vi "Add Process.vi"(8 "error in (no error)":errorcluster, 10 "Process":refnum<class "Process.lvclass">, 11 "Application In":refnum<class "Application.lvclass">) -> (0 "error out":errorcluster, 3 "Application Out":refnum<class "Application.lvclass">)   [LabVIEW 2020, in "Application.lvclass"]
doc: "Add a process to the application. The process should be initialized before being added to the application. After adding a proess, the lifecycle of the process is owned and managed by the owning application. It is therefore not necessary to Start, Stop, or Clear added processes through the lifecycle of the application."
uses:
  Application.lvclass
  C:/git/astemes-triarc-framework/source/Framework/Process/Process.lvclass
  Process/Process.lvclass
  C:/git/astemes-triarc-framework/source/Framework/Logging/Logging.lvclass
  Process/Public/Lifecycle/Lifecycle State.ctl
  Process/Process.lvclass/Process.ctl
  Application.lvclass/Application.ctl
  Synchronous Request Callback/Synchronous Request Callback.lvclass/Synchronous Request Callback.ctl
  Get Process.vi
  Process/Private/SubVIs/Handle Debug Data.vi
  <vilib>/Utility/error.llb/Clear Errors.vi
  Private/Retrieve Process from App.vi
  Private/Parse Process Name.vi
  Private/Get Process from Map.vi
  Logging/Log Debug.vi
  <vilib>/AdvancedString/1D String Array to Delimited String.vi
  <vilib>/Utility/High Resolution Relative Seconds.vi
  Process/Protected/Messaging/Request Message.vi
  <vilib>/AdvancedString/Delimited String to 1D String Array.vi
  Synchronous Request Callback/Create.vi
  Process/Protected/Messaging/Async Request Message.vi
  Synchronous Request Callback/Synchronous Request Callback.lvclass
  C:/git/astemes-triarc-framework/source/Framework/Callback/Callback.lvclass
  <vilib>/Utility/error.llb/Error Cluster From Error Code.vi
  Process/Private/SubVIs/Wait for Response Message.vi
  <vilib>/ErrorRing/Error Ring.xnode
  Callback/Callback.lvclass
  Logging/Logging.lvclass
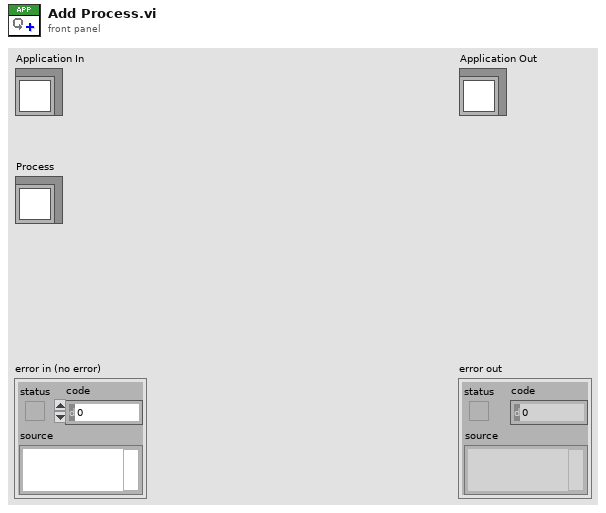
[diagram p1: front panel]
types:
  T1 = typedef "Process.lvclass/Lifecycle State.ctl" = enum16{"Uninitialized", "Initialized", "Started", "Running", "Stopped", "Finished"}
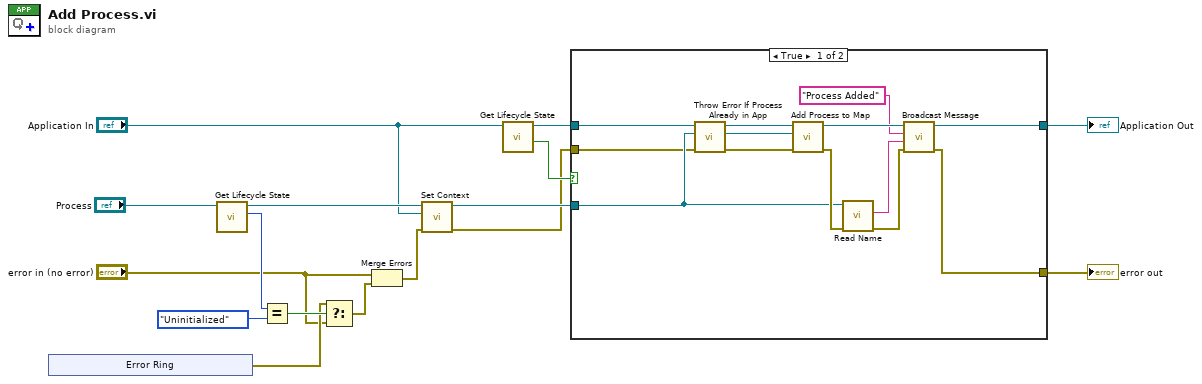
[diagram p0: block diagram]
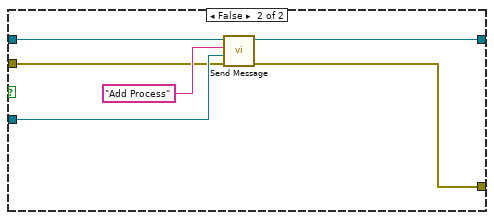
[diagram p2: hidden frame]
diagram:
  n1 = xnode "Error Ring"() -> ("error out"=w10:errorcluster)
  n2 = call "Get Lifecycle State.vi"("Process In"="Process") -> ("Lifecycle State"=w13:T1, "Process Out"=w6:refnum<class "Process.lvclass">)  [unwired: 7 in, 2 out]
  n3 = Equal?(x=w13, y=Lifecycle_State."Uninitialized" ("Lifecycle State")) -> (x = y?=w12:bool)
  n4 = Select(t=w10, s=w12, f="error in (no error)") -> (s? t:f=w11:errorcluster)
  n5 = Merge Errors("error in (no error)", w11) -> (w3:errorcluster)
  n6 = call "Set Context.vi"("error in (no error)"=w3, "Process Context"="Application In", "Process In"=w6) -> ("error out"=w2:errorcluster, "Process Out"=w5:refnum<class "Process.lvclass">)  [unwired: 7 in]
  n7 = call "Get Lifecycle State.vi"("Process In"="Application In") -> ("In Process Loop?"=w7:bool, "Process Out"=w4:refnum<class "Application.lvclass">)  [unwired: 7 in, 2 out]
  n8 = case shown="True" w7 {
    tunnel: [w28 w34] -> w16
    tunnel: [w23 w33] -> w15
    tunnel: w5 -> [w21 w32]
    tunnel: w4 -> [w22 w31]
    tunnel: w2 -> [w20 w30]
    frame True {
      n9 = call "Throw Error If Process Already in App.vi"("error in (no error)"=w20, "Process In"=w21, "Application In"=w22) -> ("error out"=w17:errorcluster, "Process Out"=w18:refnum<class "Process.lvclass">, "Application Out"=w19:refnum<class "Application.lvclass">)  [unwired: 6 in]
      n10 = call "Add Process to Map.vi"("error in (no error)"=w17, "Process Out"=w18, "Application In"=w19) -> ("error out"=w26:errorcluster, "Application Out"=w29:refnum<class "Application.lvclass">)  [unwired: 7 in]
      n11 = call "Read Name.vi"("error in (no error)"=w26, "Process In"=w21) -> ("error out"=w25:errorcluster, "Qualified Name"=w24:string)  [unwired: 6 in, 2 out]
      n12 = call-dynamic "Broadcast Message.vi"("error in (no error)"=w25, "Message Data"=w24, "Message"="Process Added", "Process In"=w29) -> ("error out"=w23:errorcluster, "Process Out"=w28:refnum<class "Application.lvclass">)  [unwired: 6 in]
    }
    frame False {
      n13 = call "Send Message.vi"("error in (no error)"=w30, "Message Data"=w32, "Message"="Add Process", "Process In"=w31) -> ("error out"=w33:errorcluster, "Process Out"=w34:refnum<class "Application.lvclass">)  [unwired: 6 in]
    }
  }
  "error out" <- w15
  "Application Out" <- w16
